vi "output.vi"(8 "error in":errorcluster, 10 "data table in":T1, 11 "Daqmx Module runtime in":refnum<class "DAQmx Module Runtime.lvclass">) -> (0 "error out":errorcluster, 2 "data table out":T1, 3 "Daqmx Module runtime out":refnum<class "DAQmx Module Runtime.lvclass">)   [LabVIEW 2015, in "DAQmx Module Runtime.lvclass"]
doc: "Provides an interface for writing data to a module at runtime. While this interface performs no operations, a child should provide an override which may write to any open sessions, references, or interfaces."
uses:
  DAQmx Module Runtime.lvclass
  <vilib>/NI/Tag Bus/table/data table.ctl
  DAQmx Module Runtime.lvclass/DAQmx Module Runtime.ctl
  <vilib>/NI/Tag Bus/table/data polymorphs/read many/read Doubles.vi
  <vilib>/DAQmx/write.llb/DAQmx Write (Analog 1D DBL NChan 1Samp).vi
  <vilib>/NI/Tag Bus/table/data polymorphs/read many/read Booleans.vi
  <vilib>/DAQmx/write.llb/DAQmx Write (Digital 1D Bool NChan 1Samp 1Line).vi
  <vilib>/DAQmx/write.llb/DAQmx Write (Counter 1D Frequency NChan 1Samp).vi
  <vilib>/DAQmx/miscellaneous.llb/DAQmx Fill In Error Info.vi
  <vilib>/NI/Tag Bus/table/data table.lvlib
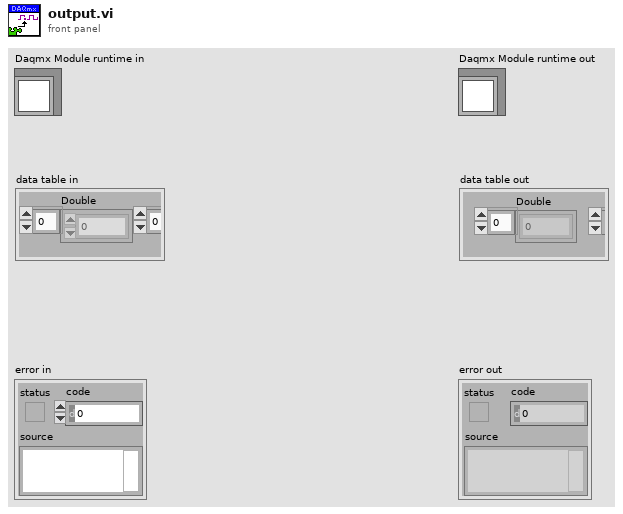
[diagram p1: front panel]
types:
  T1 = typedef "tag bus.lvlib/data table.lvlib/data table.ctl" = cluster{"Double":dbl[], "Single":sgl[], "I64":i64[], "I32":i32[], "I16":i16[], "I8":i8[], "U64":u64[], "U32":u32[], "U16":u16[], "U8":u8[], "Boolean":bool[], "String":string[], "Array of Double":cluster{"DBL Array":dbl[]}[], "Array of Single":cluster{"SGL Array":sgl[]}[], "Array of I64":cluster{"I64 Array":i64[]}[], "Array of I32":cluster{"I32 Array":i32[]}[], "Array of I16":cluster{"I16 Array":i16[]}[], "Array of I8":cluster{"I8 Array":i8[]}[], "Array of U64":cluster{"U64 Array":u64[]}[], "Array of U32":cluster{"U32 Array":u32[]}[], "Array of U16":cluster{"U16 Array":u16[]}[], "Array of U8":cluster{"U8 Array":u8[]}[], "Array of Boolean":cluster{"Boolean Array":bool[]}[], "Array of String":cluster{"String Array":string[]}[]}
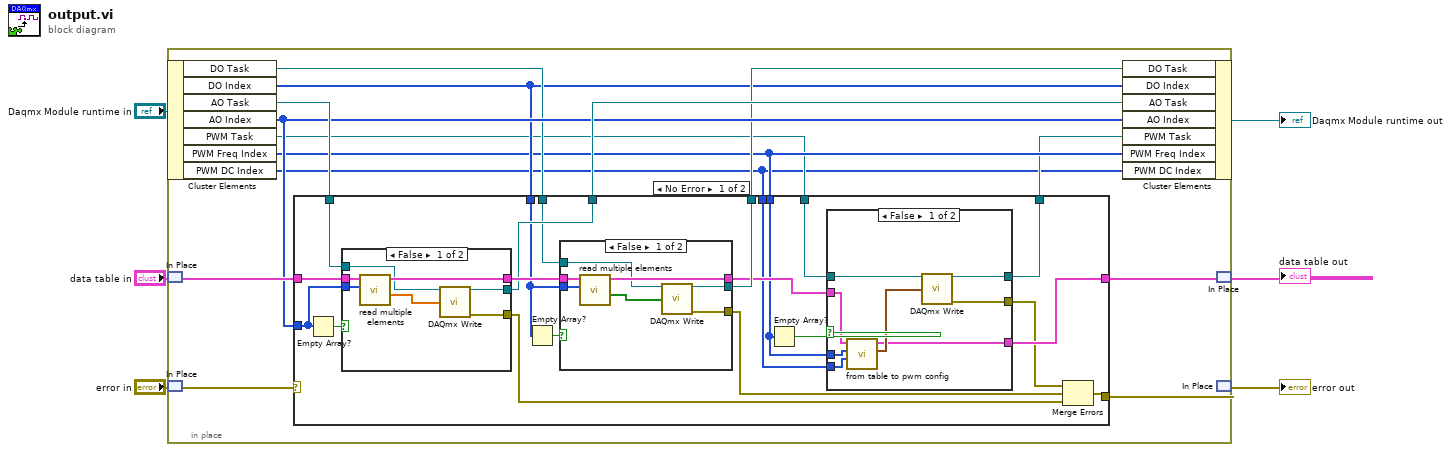
[diagram p0: block diagram]
diagram:
  n1 = in-place {
    n2 = in-place-cluster #1("Daqmx Module runtime in") -> ("DO Task"=w14:refnum<k21>, "DO Index"=w12:i32[], "AO Task"=w19:refnum<k21>, "AO Index"=w15:i32[], "PWM Task"=w9:refnum<k21>, "PWM Freq Index"=w10:i32[], "PWM DC Index"=w7:i32[])
    n3 = in-place-match #2("data table in") -> (w20:T1)
    n4 = in-place-match #3("error in") -> (w11:errorcluster)
    n5 = case shown="No Error" w11 {
      selector: w11 -> [_ w71]
      tunnel: w20 -> [w41 w72]
      tunnel: w19 -> [w40 w74]
      tunnel: [w32 w74] -> w18
      tunnel: [w26 w72] -> w17
      tunnel: [w25 w71] -> w16
      tunnel: w15 -> [w37 _]
      tunnel: w14 -> [w31 w73]
      tunnel: [w35 w73] -> w13
      tunnel: w12 -> [w30 _]
      tunnel: w10 -> [w22 _]
      tunnel: w9 -> [w28 w70]
      tunnel: [w27 w70] -> w8
      tunnel: w7 -> [w21 _]
      frame No Error {
        n6 = Empty Array?(array=w37) -> (empty?=w36:bool)
        n7 = case shown="False" w36 {
          tunnel: w41 -> [w67 w69]
          tunnel: [w66 w69] -> w39
          tunnel: w40 -> [w65 w68]
          tunnel: [w64 w68] -> w32
          tunnel: w37 -> [w62 _]
          tunnel: [w61 _] -> w34
          frame False {
            n8 = call-poly <vilib>:"read multiple elements.vi"("indices"=w62, "data table in"=w67) -> ("values"=w63:dbl[], "data table out"=w66:T1)  [unwired: 8 in]
            n9 = call-poly <vilib>:"DAQmx Write.vi"("task/channels in"=w65, "data"=w63) -> ("task out"=w64:refnum<k21>, "error out"=w61:errorcluster)  [unwired: 11 in, 1 out]
          }
          frame True {
          }
        }
        n10 = Empty Array?(array=w30) -> (empty?=w38:bool)
        n11 = case shown="False" w38 {
          tunnel: w39 -> [w58 w59]
          tunnel: [w57 w59] -> w29
          tunnel: w31 -> [w56 w60]
          tunnel: [w55 w60] -> w35
          tunnel: w30 -> [w54 _]
          tunnel: [w53 _] -> w33
          frame False {
            n12 = call-poly <vilib>:"read multiple elements.vi"("indices"=w54, "data table in"=w58) -> ("values"=w52:bool[], "data table out"=w57:T1)  [unwired: 8 in]
            n13 = call-poly <vilib>:"DAQmx Write.vi"("task/channels in"=w56, "data"=w52) -> ("task out"=w55:refnum<k21>, "error out"=w53:errorcluster)  [unwired: 11 in, 1 out]
          }
          frame True {
          }
        }
        n14 = Empty Array?(array=w22) -> (empty?=w23:bool)
        n15 = case shown="False" w23 {
          tunnel: w29 -> [w46 w50]
          tunnel: [w42 w50] -> w26
          tunnel: w28 -> [w49 w51]
          tunnel: [w48 w51] -> w27
          tunnel: w22 -> [w44 _]
          tunnel: [w47 _] -> w24
          tunnel: w21 -> [w43 _]
          frame False {
            n16 = call "from table to pwm config.vi"("PWM DC Index"=w43, "PWM Freq Index"=w44, "data table in"=w46) -> ("PWM Config Array Out"=w45:cluster{"duty cycle":dbl, "frequency":dbl}[], "data table out"=w42:T1)  [unwired: 7 in]
            n17 = call-poly <vilib>:"DAQmx Write.vi"("task/channels in"=w49, "data"=w45) -> ("task out"=w48:refnum<k21>, "error out"=w47:errorcluster)  [unwired: 11 in, 1 out]
          }
          frame True {
          }
        }
        n18 = Merge Errors(w24, w33, w34) -> (w25:errorcluster)
      }
      frame Error {
      }
    }
    n19 = in-place-cluster #1("DO Task"=w13, "DO Index"=w12, "AO Task"=w18, "AO Index"=w15, "PWM Task"=w8, "PWM Freq Index"=w10, "PWM DC Index"=w7) -> (→"Daqmx Module runtime out":refnum<class "DAQmx Module Runtime.lvclass">)
    n20 = in-place-match #2(w17) -> (→"data table out":T1)
    n21 = in-place-match #3(w16) -> (→"error out":errorcluster)
  }
